vi "optical_grab2.vi"() -> ()   [LabVIEW 2025]
uses:
  <vilib>/vision/driver/NI_Vision_Acquisition_Software.lvlib
panel:
  in  "Image Type (IMAQ)":T1 items=["Grayscale (U8)", "Grayscale (I16)", "Grayscale (SGL)", "Complex (CSG)", "RGB (U32)", "HSL (U32)", "RGB (U64)", "Grayscale (U16)"]
  out "Image Type Out":T1 items=["Grayscale (U8)", "Grayscale (I16)", "Grayscale (SGL)", "Complex (CSG)", "RGB (U32)", "HSL (U32)", "RGB (U64)", "Grayscale (U16)"]
  out "Image Preview":T2(plugin-control)
  out "error out":errorcluster
  out "FPS":u32
  in  "Output Folder":path=path "../data/raw/test_6"
  in  "Stop":bool
  in  "Camera Name":refnum<k21> caption="IMAQdx Session"
  # "-> Grab VI ->"
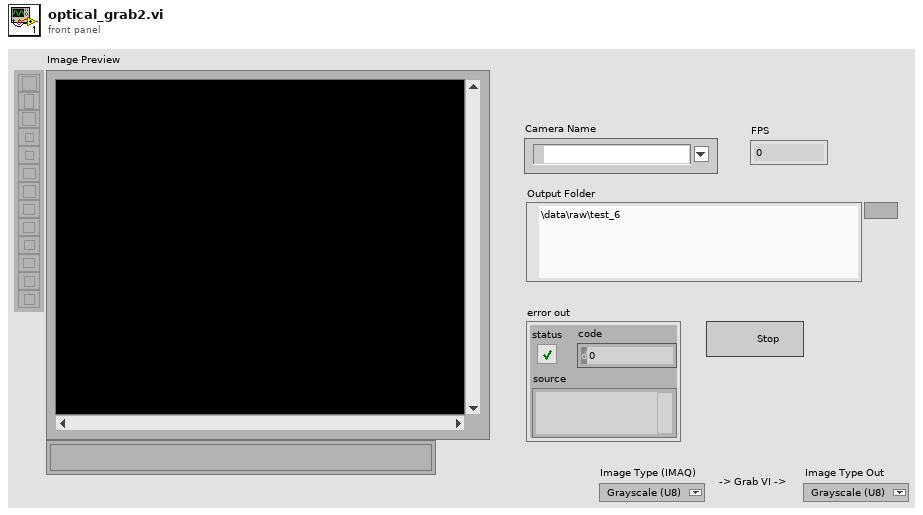
[diagram p1: front panel]
types:
  T1 = typedef "Image Type" = u32
  T2 = typedef "IMAQ Image.ctl" = refnum<image>
  T3 = typedef "IMAQdx.ctl" = refnum<k21>
  T4 = enum16{"big-endian, network order", "native, host order", "little-endian"}
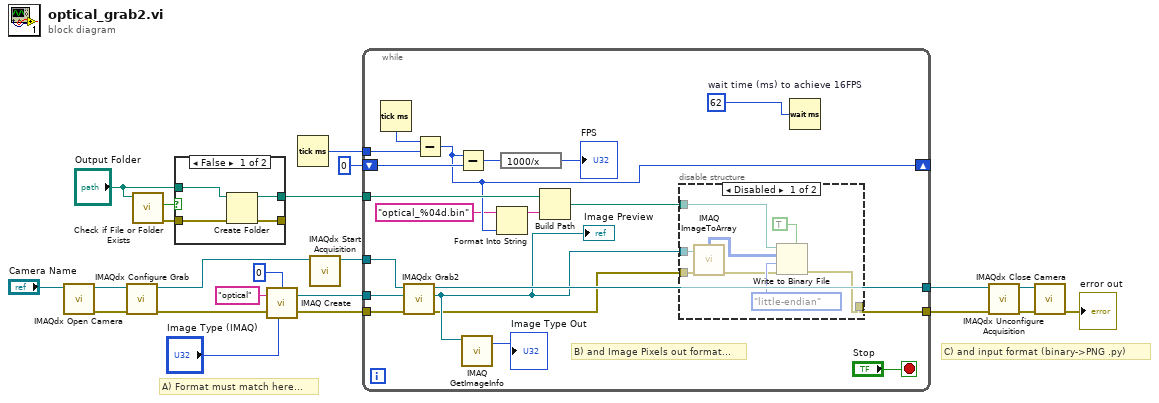
[diagram p0: block diagram]
diagram:
  # "C) and input format (binary->PNG .py)"
  # "A) Format must match here..."
  n1 = call <vilib>:"IMAQdx Open Camera.vi"("Session In"="Camera Name") -> ("error out"=w8:errorcluster, "Session Out"=w10:T3)  [unwired: 9 in]
  n2 = call <vilib>:"IMAQdx Configure Grab.vi"("error in"=w8, "Session In"=w10) -> ("error out"=w7:errorcluster, "Session Out"=w9:T3)  [unwired: 8 in]
  n3 = call <vilib>:"Check if File or Folder Exists.vi"("path"="Output Folder") -> ("error out"=w20:errorcluster, "file or folder exists?"=w22:bool)  [unwired: 8 in, 1 out]
  n4 = case shown="False" w22 {
    tunnel: "Output Folder" -> [w26 w28]
    tunnel: [w25 w28] -> w19
    tunnel: w20 -> [w24 w27]
    tunnel: [w23 w27] -> _
    frame False {
      n5 = Create Folder(path (use dialog)=w26, error in=w24) -> (created path=w25:path, error out=w23:errorcluster)  [unwired: 1 in, 1 out]
    }
    frame True {
    }
  }
  n6 = call "IMAQ Create"("Border Size"=0, "Image Name"="optical", "Image Type"="Image Type (IMAQ)", "error in (no error)"=w7) -> ("New Image"=w1:T2, "error out"=w11:errorcluster)  [unwired: 1 in]
  n7 = Tick Count (ms)() -> (millisecond timer value=w18:u32)
  n8 = call <vilib>:"IMAQdx Start Acquisition.vi"("Session In"=w9) -> ("Session Out"=w12:T3)  [unwired: 9 in, 1 out]
  n9 = while {
    tunnel: w19 -> [w48]
    tunnel: w18 -> [w46]
    shift-right: [w44] -> _
    shift-left: u32 0 -> [w45]
    tunnel: w12 -> [w40]
    tunnel: w1 -> [w39]
    tunnel: w11 -> [w38]
    tunnel: [w33] -> w6
    tunnel: [w36] -> w3
    stop <- "Stop" stop-if-true
    w29 = u32 62  # wait time (ms) to achieve 16FPS
    # "B) and Image Pixels out format..."
    n10 = Tick Count (ms)() -> (millisecond timer value=w47:u32)
    n11 = call <vilib>:"IMAQdx Grab2.vi"("error in"=w38, "Image In"=w39, "Session In"=w40) -> ("error out"=w30:errorcluster, "Image Out"=w31:T2, "Session Out"=w33:T3)  [unwired: 5 in, 1 out]
    "Image Preview" <- w31
    n12 = Subtract(x=w47, y=w46) -> (x-y=w44:u32)
    n13 = Subtract(x=w44, y=w45) -> (x-y=w35:u32)
    n14 = call "IMAQ GetImageInfo"("Image"=w31) -> ("Image Type"=→"Image Type Out":T1)  [unwired: 3 in, 7 out]
    n15 = Format Into String(format string="optical_%04d.bin", w44) -> (resulting string=w43:string)  [unwired: 2 in, 1 out]
    n16 = expression code="1000/x"(w35) -> (→"FPS":u32)
    n17 = Build Path(base path=w48, name or relative path=w43) -> (appended path=w37:path)
    n18 = disable-structure shown="Disabled" {
      disable-tunnel: w37 -> [w56 _]
      disable-tunnel: [w55 w57] -> w36
      disable-tunnel: w31 -> [w52 _]
      disable-tunnel: w30 -> [w51 w57]
      frame Disabled {
        n19 = call "IMAQ ImageToArray"("error in (no error)"=w51, "Image"=w52) -> ("error out"=w50:errorcluster, "Image Pixels (U8)"=w49:u8[][])  [unwired: 2 in, 3 out]
        n20 = Write to Binary File(file (use dialog)=w56, data=w49, error in=w50, 5:TRUE, 9:T4."little-endian" ("byte order (0:big-endian, network order)")) -> (error out=w55:errorcluster)  [unwired: 1 in, 2 out]
      }
      frame Enabled {
      }
    }
    n21 = Wait (ms)(milliseconds to wait=w29) -> ()  [unwired: 1 out]
  }
  n22 = call <vilib>:"IMAQdx Unconfigure Acquisition.vi"("error in"=w3, "Session In"=w6) -> ("error out"=w4:errorcluster, "Session Out"=w5:T3)  [unwired: 8 in]
  n23 = call <vilib>:"IMAQdx Close Camera.vi"("error in"=w4, "Session In"=w5) -> ("error out"=→"error out":errorcluster)  [unwired: 9 in]
